vi "test access bearer token.vi"(8 "error in (no error)":errorcluster) -> (0 "error out":errorcluster, 3 "body":string)   [LabVIEW 2020, in "MCP Server tests.lvlib"]
doc: "Bearer token. A second MCP server is started on port 37062 with Access token = \"test-token-62\". tools/list without an Authorization header and with a wrong token is answered with HTTP 401, WWW-Authenticate: Bearer and the JSON-RPC error {\"jsonrpc\":\"2.0\",\"id\":null,\"error\":{\"code\":-32600,\"message\":\"Unauthorized: missing or invalid bearer token.\"}}; with \"Authorization: bearer test-token-62\" (lower-case scheme) and with the header name in lower case it is answered normally (200 and a result). The token never appears in any response. The server is stopped afterwards."
uses:
  MCP Server tests.lvlib
  <vilib>/addons/_JKI Toolkits/Caraya/classes/Test/Test.lvclass
  src/MCP Server/MCP Server.lvlib
  <vilib>/addons/_JKI Toolkits/Caraya/classes/Assert/Assert.lvclass
panel:
  out "lookup error":errorcluster
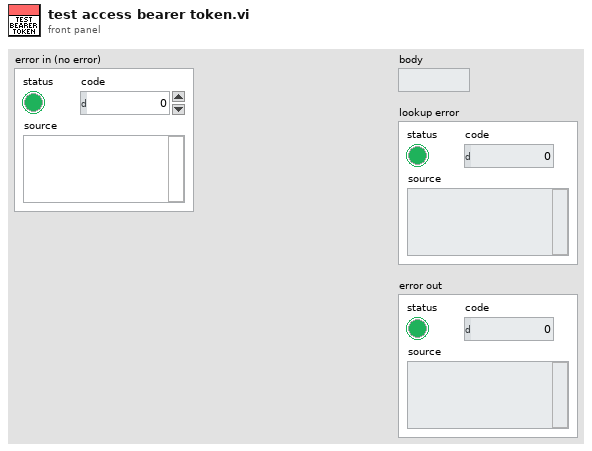
[diagram p1: front panel]
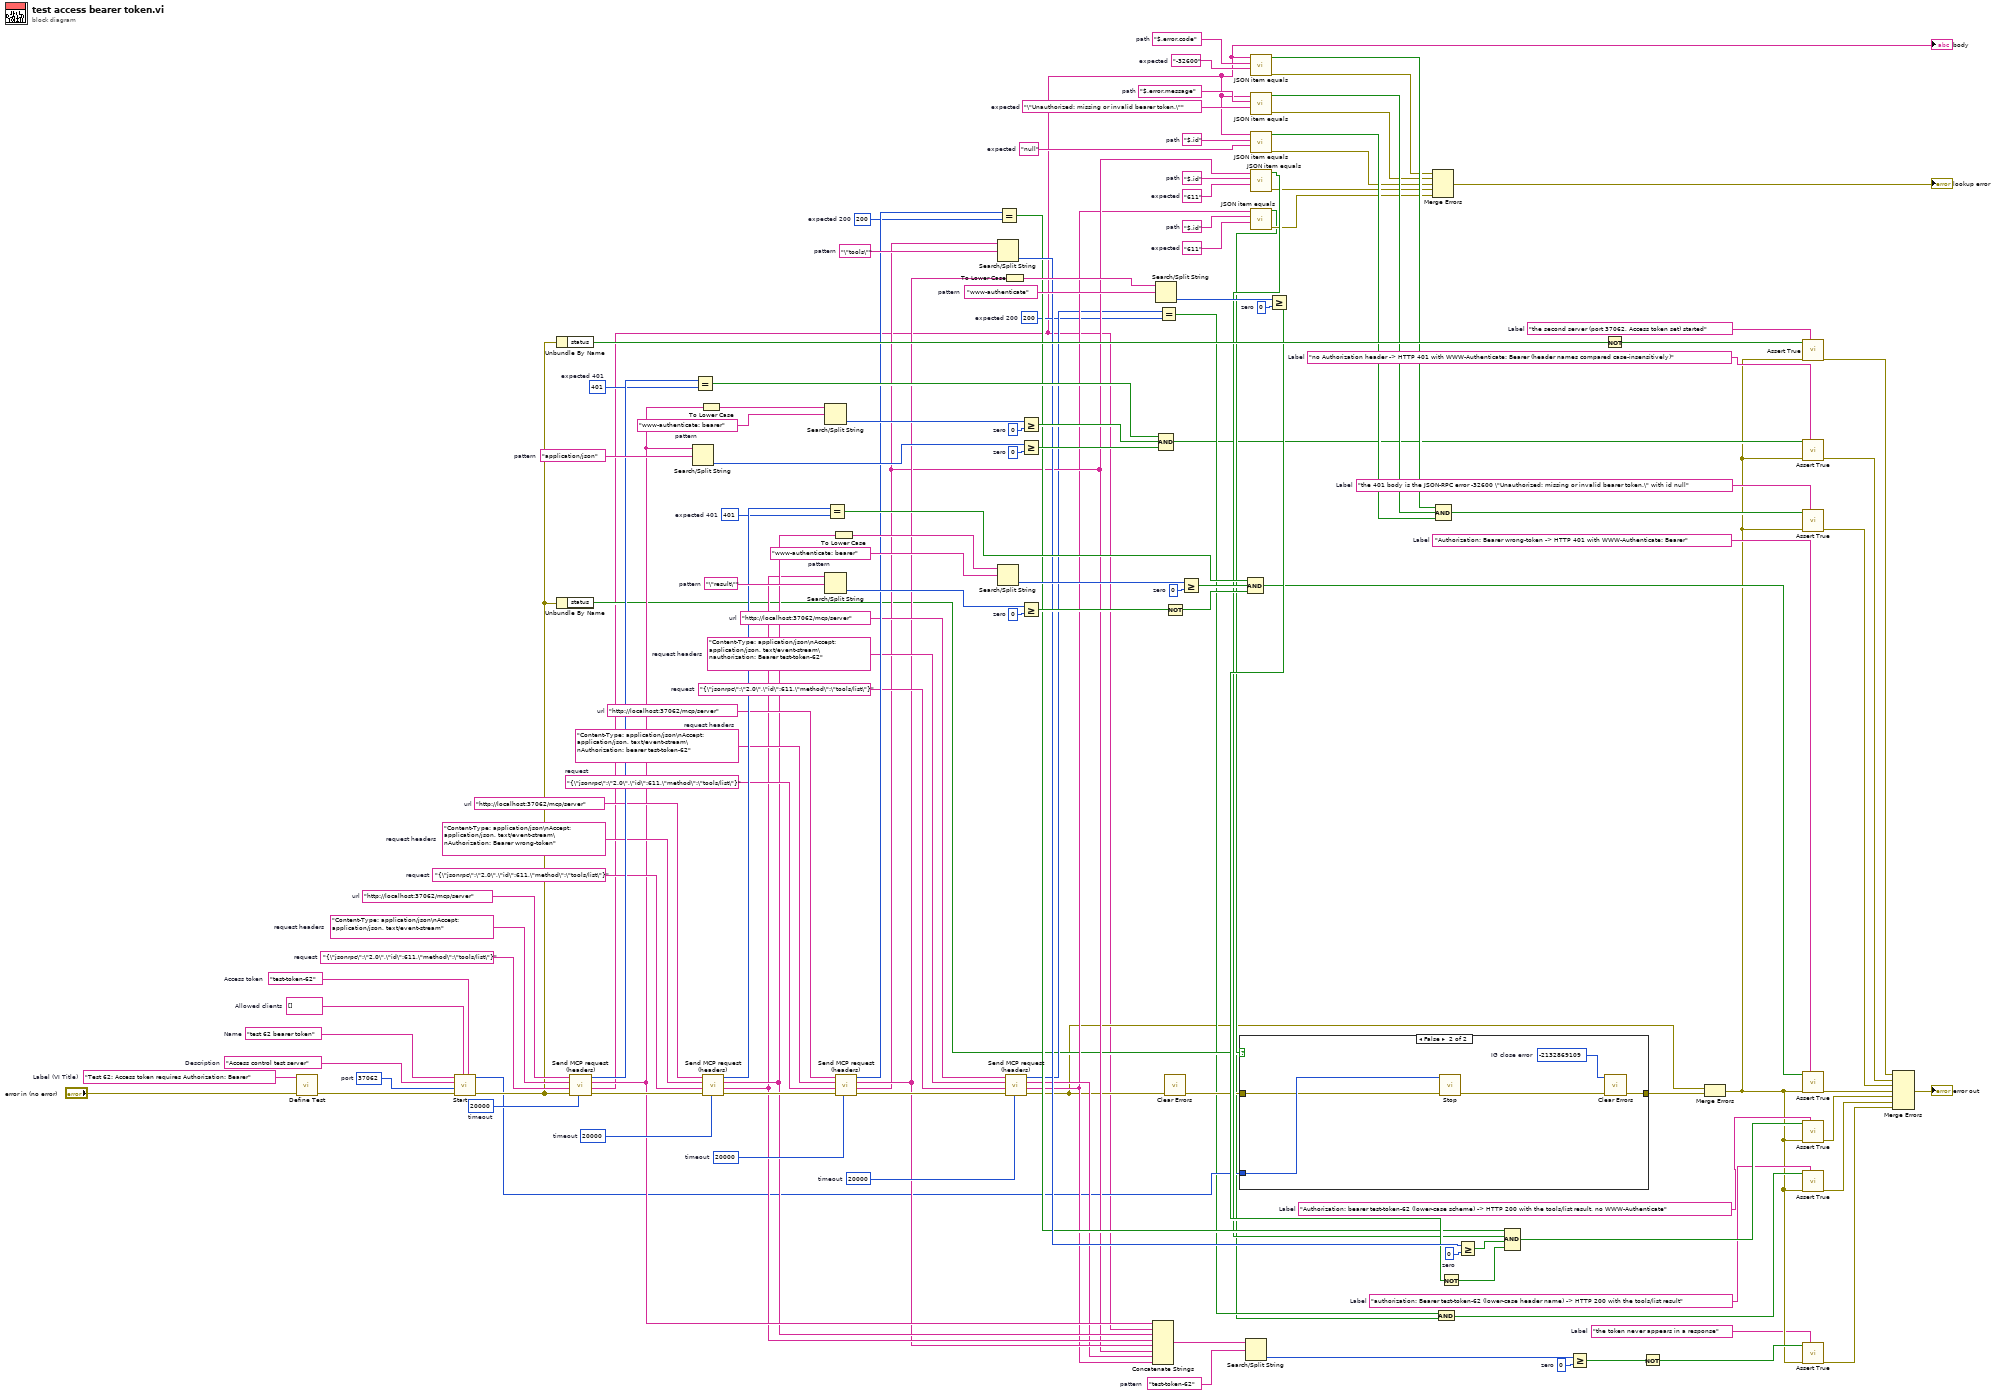
[diagram p0: block diagram]
diagram:
  w57 = "Content-Type: application/json\nAccept: application/json, text/event-stream\nauthorization: Bearer test-token-62"  # request headers
  w78 = "Content-Type: application/json\nAccept: application/json, text/event-stream\nAuthorization: bearer test-token-62"  # request headers
  w96 = "Content-Type: application/json\nAccept: application/json, text/event-stream\nAuthorization: Bearer wrong-token"  # request headers
  w122 = "Content-Type: application/json\nAccept: application/json, text/event-stream"  # request headers
  w11 = "the token never appears in a response"  # Label
  w14 = "authorization: Bearer test-token-62 (lower-case header name) -> HTTP 200 with the tools/list result"  # Label
  w16 = "Authorization: bearer test-token-62 (lower-case scheme) -> HTTP 200 with the tools/list result, no WWW-Authenticate"  # Label
  w18 = "Authorization: Bearer wrong-token -> HTTP 401 with WWW-Authenticate: Bearer"  # Label
  w20 = "the 401 body is the JSON-RPC error -32600 \"Unauthorized: missing or invalid bearer token.\" with id null"  # Label
  w22 = "no Authorization header -> HTTP 401 with WWW-Authenticate: Bearer (header names compared case-insensitively)"  # Label
  w24 = "the second server (port 37062, Access token set) started"  # Label
  w34 = 0  # zero
  w38 = "test-token-62"  # pattern
  w41 = "611"  # expected
  w42 = "$.id"  # path
  w36 = 200  # expected 200
  w64 = 0  # zero
  w72 = "www-authenticate"  # pattern
  w68 = 0  # zero
  w74 = "\"tools\""  # pattern
  w70 = "611"  # expected
  w71 = "$.id"  # path
  w66 = 200  # expected 200
  w88 = 0  # zero
  w92 = "\"result\""  # pattern
  w84 = 0  # zero
  w90 = "www-authenticate: bearer"  # pattern
  w86 = 401  # expected 401
  w108 = "null"  # expected
  w109 = "$.id"  # path
  w110 = "\"Unauthorized: missing or invalid bearer token.\""  # expected
  w111 = "$.error.message"  # path
  w112 = "-32600"  # expected
  w113 = "$.error.code"  # path
  w114 = 0  # zero
  w118 = "application/json"  # pattern
  w104 = 0  # zero
  w116 = "www-authenticate: bearer"  # pattern
  w106 = 401  # expected 401
  w55 = 20000  # timeout
  w56 = "{\"jsonrpc\":\"2.0\",\"id\":611,\"method\":\"tools/list\"}"  # request
  w58 = "http://localhost:37062/mcp/server"  # url
  w76 = 20000  # timeout
  w77 = "{\"jsonrpc\":\"2.0\",\"id\":611,\"method\":\"tools/list\"}"  # request
  w79 = "http://localhost:37062/mcp/server"  # url
  w94 = 20000  # timeout
  w95 = "{\"jsonrpc\":\"2.0\",\"id\":611,\"method\":\"tools/list\"}"  # request
  w97 = "http://localhost:37062/mcp/server"  # url
  w120 = 20000  # timeout
  w121 = "{\"jsonrpc\":\"2.0\",\"id\":611,\"method\":\"tools/list\"}"  # request
  w123 = "http://localhost:37062/mcp/server"  # url
  w125 = "test-token-62"  # Access token
  w126 = string[] []  # Allowed clients
  w128 = u16 37062  # port
  w129 = "Access control test server"  # Description
  w130 = "test 62 bearer token"  # Name
  w132 = "Test 62: Access token requires Authorization: Bearer"  # Label (VI Title)
  n1 = call <vilib>:"Define Test.vi"("error in (no error)"="error in (no error)", "Label (VI Title)"=w132) -> ("error out"=w127:errorcluster)  [unwired: 8 in, 1 out]
  n2 = call "Start.vi"("Access token"=w125, "Allowed clients"=w126, "error in (no error)"=w127, "HTTP Port (36987)"=w128, "Description"=w129, "Name"=w130) -> ("error out"=w119:errorcluster, "server id out"=w33:i32)  [unwired: 3 in, 1 out]
  n3 = Unbundle By Name(w119) -> ("status"=w124:bool)
  n4 = Unbundle By Name(w119) -> ("status"=w31:bool)
  n5 = call "Send MCP request (headers).vi"("timeout (10000)"=w120, "error in (no error)"=w119, "request"=w121, "request headers"=w122, "url"=w123) -> ("error out"=w93:errorcluster, "response"=w3:string, "headers"=w53:string, "status code"=w107:i32)  [unwired: 3 in]
  "body" <- w3
  n6 = Search/Split String(string=w53, search string/char (-)=w118) -> (offset of match=w115:i32)  [unwired: 1 in, 2 out]
  n7 = Equal?(x=w107, y=w106) -> (x = y?=w100:bool)
  n8 = To Lower Case(string=w53) -> (all lower case string=w117:string)
  n9 = call "Send MCP request (headers).vi"("timeout (10000)"=w94, "error in (no error)"=w93, "request"=w95, "request headers"=w96, "url"=w97) -> ("error out"=w75:errorcluster, "response"=w51:string, "headers"=w52:string, "status code"=w87:i32)  [unwired: 3 in]
  n10 = Search/Split String(string=w117, search string/char (-)=w116) -> (offset of match=w105:i32)  [unwired: 1 in, 2 out]
  n11 = Search/Split String(string=w51, search string/char (-)=w92) -> (offset of match=w89:i32)  [unwired: 1 in, 2 out]
  n12 = Equal?(x=w87, y=w86) -> (x = y?=w82:bool)
  n13 = To Lower Case(string=w52) -> (all lower case string=w91:string)
  n14 = call "Send MCP request (headers).vi"("timeout (10000)"=w76, "error in (no error)"=w75, "request"=w77, "request headers"=w78, "url"=w79) -> ("error out"=w54:errorcluster, "response"=w49:string, "headers"=w50:string, "status code"=w67:i32)  [unwired: 3 in]
  n15 = Search/Split String(string=w49, search string/char (-)=w74) -> (offset of match=w69:i32)  [unwired: 1 in, 2 out]
  n16 = Search/Split String(string=w91, search string/char (-)=w90) -> (offset of match=w85:i32)  [unwired: 1 in, 2 out]
  n17 = Equal?(x=w67, y=w66) -> (x = y?=w62:bool)
  n18 = To Lower Case(string=w50) -> (all lower case string=w73:string)
  n19 = call "Send MCP request (headers).vi"("timeout (10000)"=w55, "error in (no error)"=w54, "request"=w56, "request headers"=w57, "url"=w58) -> ("error out"=w27:errorcluster, "response"=w43:string, "headers"=w48:string, "status code"=w37:i32)  [unwired: 3 in]
  n20 = Greater Or Equal?(x=w105, y=w104) -> (x >= y?=w99:bool)
  n21 = Greater Or Equal?(x=w115, y=w114) -> (x >= y?=w98:bool)
  n22 = Greater Or Equal?(x=w89, y=w88) -> (x >= y?=w83:bool)
  n23 = Concatenate Strings(w53, w3, w52, w51, w50, w49, w48, w43) -> (w39:string)
  n24 = Search/Split String(string=w73, search string/char (-)=w72) -> (offset of match=w65:i32)  [unwired: 1 in, 2 out]
  n25 = Equal?(x=w37, y=w36) -> (x = y?=w30:bool)
  n26 = Compound Arithmetic op=AND(w100, w99, w98) -> (w23:bool)
  n27 = Not(x=w83) -> (.not. x?=w80:bool)
  n28 = call <vilib>:"Clear Errors.vi"("error in (no error)"=w27) -> ("error out"=w32:errorcluster)  [unwired: 5 in, 1 out]
  n29 = Greater Or Equal?(x=w85, y=w84) -> (x >= y?=w81:bool)
  n30 = case shown="False" w31 {
    tunnel: w33 -> [_ w138]
    tunnel: w32 -> [w133 w137]
    tunnel: [w133 w134] -> w26
    frame True {
    }
    frame False {
      w136 = -2132869109  # IG close error
      n31 = call "Stop.vi"("error in (no error)"=w137, "id"=w138) -> ("error out"=w135:errorcluster)  [unwired: 9 in]
      n32 = call <vilib>:"Clear Errors.vi"("error in (no error)"=w135, "specific error code to clear (0: all)"=w136) -> ("error out"=w134:errorcluster)  [unwired: 4 in, 1 out]
    }
  }
  n33 = Search/Split String(string=w39, search string/char (-)=w38) -> (offset of match=w35:i32)  [unwired: 1 in, 2 out]
  n34 = Compound Arithmetic op=AND(w82, w81, w80) -> (w19:bool)
  n35 = call "JSON item equals.vi"("expected"=w112, "path"=w113, "JSON"=w3) -> ("error out"=w47:errorcluster, "equal?"=w103:bool)  [unwired: 6 in, 1 out]
  n36 = call "JSON item equals.vi"("expected"=w110, "path"=w111, "JSON"=w3) -> ("error out"=w46:errorcluster, "equal?"=w102:bool)  [unwired: 6 in, 1 out]
  n37 = call "JSON item equals.vi"("expected"=w108, "path"=w109, "JSON"=w3) -> ("error out"=w45:errorcluster, "equal?"=w101:bool)  [unwired: 6 in, 1 out]
  n38 = call "JSON item equals.vi"("expected"=w70, "path"=w71, "JSON"=w49) -> ("error out"=w44:errorcluster, "equal?"=w61:bool)  [unwired: 6 in, 1 out]
  n39 = call "JSON item equals.vi"("expected"=w41, "path"=w42, "JSON"=w43) -> ("error out"=w40:errorcluster, "equal?"=w29:bool)  [unwired: 6 in, 1 out]
  n40 = Greater Or Equal?(x=w65, y=w64) -> (x >= y?=w63:bool)
  n41 = Merge Errors(w47, w46, w45, w44, w40) -> (→"lookup error":errorcluster)
  n42 = Compound Arithmetic op=AND(w103, w102, w101) -> (w21:bool)
  n43 = And(x=w30, y=w29) -> (x .and. y?=w15:bool)
  n44 = Not(x=w63) -> (.not. x?=w59:bool)
  n45 = Greater Or Equal?(x=w69, y=w68) -> (x >= y?=w60:bool)
  n46 = Compound Arithmetic op=AND(w62, w61, w60, w59) -> (w17:bool)
  n47 = Greater Or Equal?(x=w35, y=w34) -> (x >= y?=w28:bool)
  n48 = Not(x=w124) -> (.not. x?=w25:bool)
  n49 = Not(x=w28) -> (.not. x?=w13:bool)
  n50 = Merge Errors(w27, w26) -> (w12:errorcluster)
  n51 = call <vilib>:"Assert True.vi"("Label"=w24, "error in (no error)"=w12, "True?"=w25) -> ("error out"=w10:errorcluster)  [unwired: 7 in, 1 out]
  n52 = call <vilib>:"Assert True.vi"("Label"=w22, "error in (no error)"=w12, "True?"=w23) -> ("error out"=w9:errorcluster)  [unwired: 7 in, 1 out]
  n53 = call <vilib>:"Assert True.vi"("Label"=w20, "error in (no error)"=w12, "True?"=w21) -> ("error out"=w8:errorcluster)  [unwired: 7 in, 1 out]
  n54 = call <vilib>:"Assert True.vi"("Label"=w18, "error in (no error)"=w12, "True?"=w19) -> ("error out"=w7:errorcluster)  [unwired: 7 in, 1 out]
  n55 = call <vilib>:"Assert True.vi"("Label"=w16, "error in (no error)"=w12, "True?"=w17) -> ("error out"=w6:errorcluster)  [unwired: 7 in, 1 out]
  n56 = call <vilib>:"Assert True.vi"("Label"=w14, "error in (no error)"=w12, "True?"=w15) -> ("error out"=w5:errorcluster)  [unwired: 7 in, 1 out]
  n57 = call <vilib>:"Assert True.vi"("Label"=w11, "error in (no error)"=w12, "True?"=w13) -> ("error out"=w4:errorcluster)  [unwired: 7 in, 1 out]
  n58 = Merge Errors(w10, w9, w8, w7, w6, w5, w4) -> (→"error out":errorcluster)
